vi "OwnFile20261012_Own20261012_GetTerminalContext.vi"() -> ()   [LabVIEW 2024]
panel:
  out "error out":errorcluster caption="错误输出"
  out "diagram_id":refnum<vi>
  out "is_source":bool
  in  "terminal_id":u32
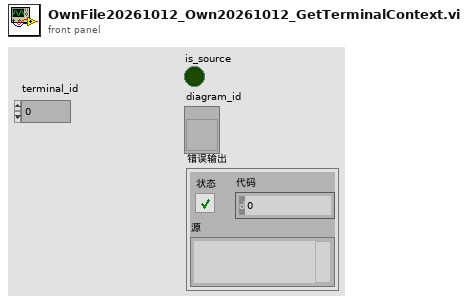
[diagram p1: front panel]
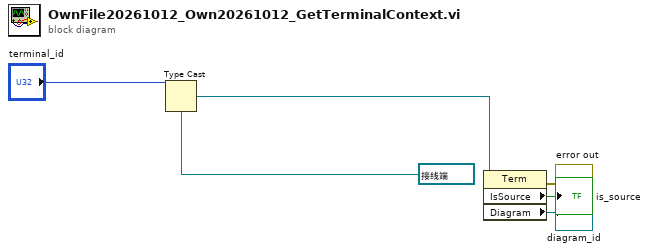
[diagram p0: block diagram]
diagram:
  n1 = Type Cast(type=refnum<vi> refnum ("引用"), x="terminal_id") -> (*(type *) &x=w4:refnum<vi>)
  n2 = property class="Term"(reference=w4) -> (error out=→"error out":errorcluster, "IsSource"=→"is_source":bool, "Diagram"=→"diagram_id":refnum<vi>)  [unwired: 1 in, 1 out]
